vi "Get Time Pair.vi"(8 "error in (no error)":errorcluster, 11 "XNET CAN RW in":refnum<class "XNET CAN RW.lvclass">) -> (0 "error out":errorcluster, 2 "Time Pair":T1, 3 "XNET CAN RW out":refnum<class "XNET CAN RW.lvclass">)   [LabVIEW 2021, in "XNET CAN RW.lvclass"]
doc: "Get a timestamp pair to correlate the current time of the CAN interface with the system time. Times are returned in TAI timescale in ns."
uses:
  XNET CAN RW.lvclass
  typedef/Time Pair.ctl
  XNET CAN RW.lvclass/XNET CAN RW.ctl
  <vilib>/xnet/xnet.llb/XNET Read (State Time Current).vi
  <vilib>/CIF Foundation/CIF Utilities/Time/Time_CIF_U.lvlib
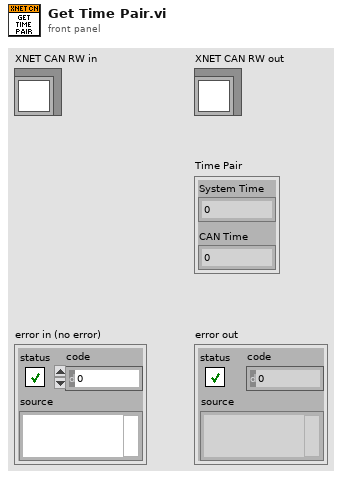
[diagram p1: front panel]
types:
  T1 = typedef "XNET CAN RW.lvclass/Time Pair.ctl" = cluster{"System Time":i64, "CAN Time":i64}
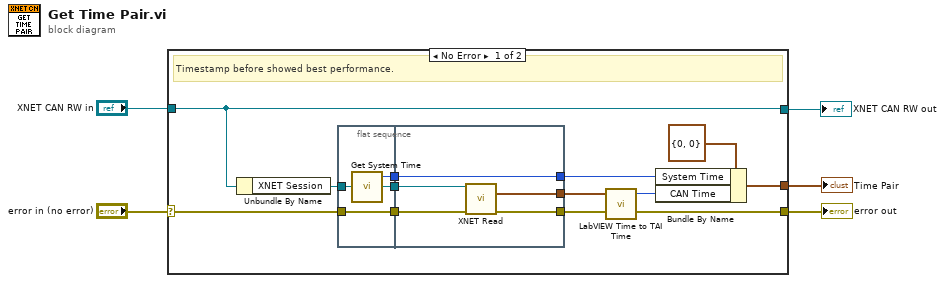
[diagram p0: block diagram]
diagram:
  n1 = case shown="No Error" "error in (no error)" {
    selector: "error in (no error)" -> [w15 w27]
    tunnel: [w13 w27] -> w4
    tunnel: [w14 w26] -> w2
    tunnel: "XNET CAN RW in" -> [w14 w26]
    tunnel: [w7 _] -> w1
    frame No Error {
      # "Timestamp before showed best performance."
      n2 = Unbundle By Name(w14) -> ("XNET Session"=w17:refnum<k21>)
      n3 = flat-sequence {
        tunnel: w15 -> [w19]
        tunnel: w17 -> [w20]
        tunnel: [w20] -> w12
        tunnel: [w19] -> w11
        tunnel: [w18] -> w10
        tunnel: w12 -> [w25]
        tunnel: w11 -> [w23]
        tunnel: w10 -> [w21]
        tunnel: [w24] -> w16
        tunnel: [w22] -> w13
        tunnel: [w21] -> w6
        frame #0 {
          n4 = call <vilib>:"Get System Time.vi"() -> ("Time (ns)"=w18:i64)  [unwired: 5 in]
        }
        frame #1 {
          n5 = call-poly <vilib>:"XNET Read.vi"("session in"=w25, "error in (no error)"=w23) -> ("local time current"=w24:timestamp, "error out"=w22:errorcluster)  [unwired: 9 in, 3 out]
        }
      }
      n6 = call <vilib>:"LabVIEW Time to TAI Time.vi"("LabVIEW Time (s)"=w16) -> ("TAI Time (ns)"=w8:i64)  [unwired: 4 in]
      n7 = Bundle By Name(cluster=T1 {"System Time"=0, "CAN Time"=0} ("Time Pair 2"), "System Time"=w6, "CAN Time"=w8) -> (w7:T1)
    }
    frame Error {
    }
  }
  "error out" <- w4
  "XNET CAN RW out" <- w2
  "Time Pair" <- w1
